vi "OwnCompat20261012_Native_SetControlLabel.vi"() -> ()   [LabVIEW 2024]
panel:
  out "error out":errorcluster caption="错误输出"
  in  "label":string
  in  "control_id":u32
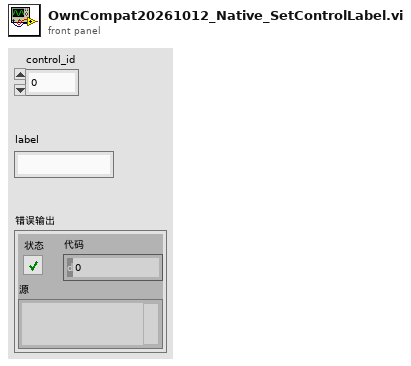
[diagram p1: front panel]
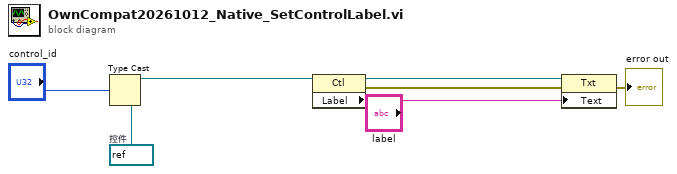
[diagram p0: block diagram]
diagram:
  w6 = refnum<vi> refnum  # 控件
  n1 = Type Cast ("强制类型转换")(type=w6, x="control_id") -> (*(type *) &x=w5:refnum<vi>)
  n2 = property on="属性节点" class="Ctl"(reference=w5) -> (error out=w2:errorcluster, "Label"=w4:refnum<vi>)  [unwired: 1 in, 1 out]
  n3 = property on="属性节点" class="Txt"(reference=w4, error in=w2, "Text"="label") -> (error out=→"error out":errorcluster)  [unwired: 1 out]
